vi "test_full_flow.vi"() -> ()   [LabVIEW 2020, in "reqwest_tests.lvlib"]
uses:
  reqwest_tests.lvlib
  <vilib>/addons/_JKI Toolkits/Caraya/classes/Assert/Assert.lvclass
  <vilib>/addons/_JKI Toolkits/Caraya/classes/Test/Test.lvclass
  ClientBuilder/ClientBuilder.lvclass
  Client/Client.lvclass
  Headers/Headers.lvclass
  Request/Request.lvclass
panel:
  out "is_complete":bool
  out "string_value":string
  in  "error in (no error)":errorcluster
  out "error out":errorcluster
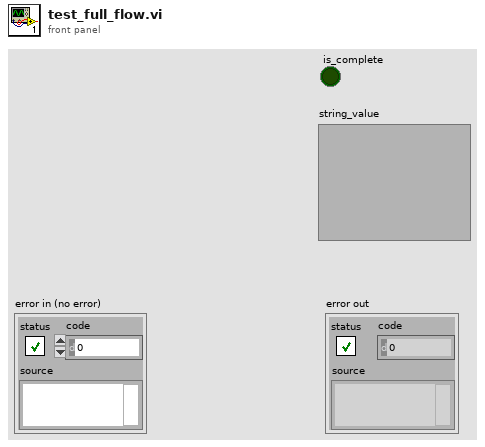
[diagram p1: front panel]
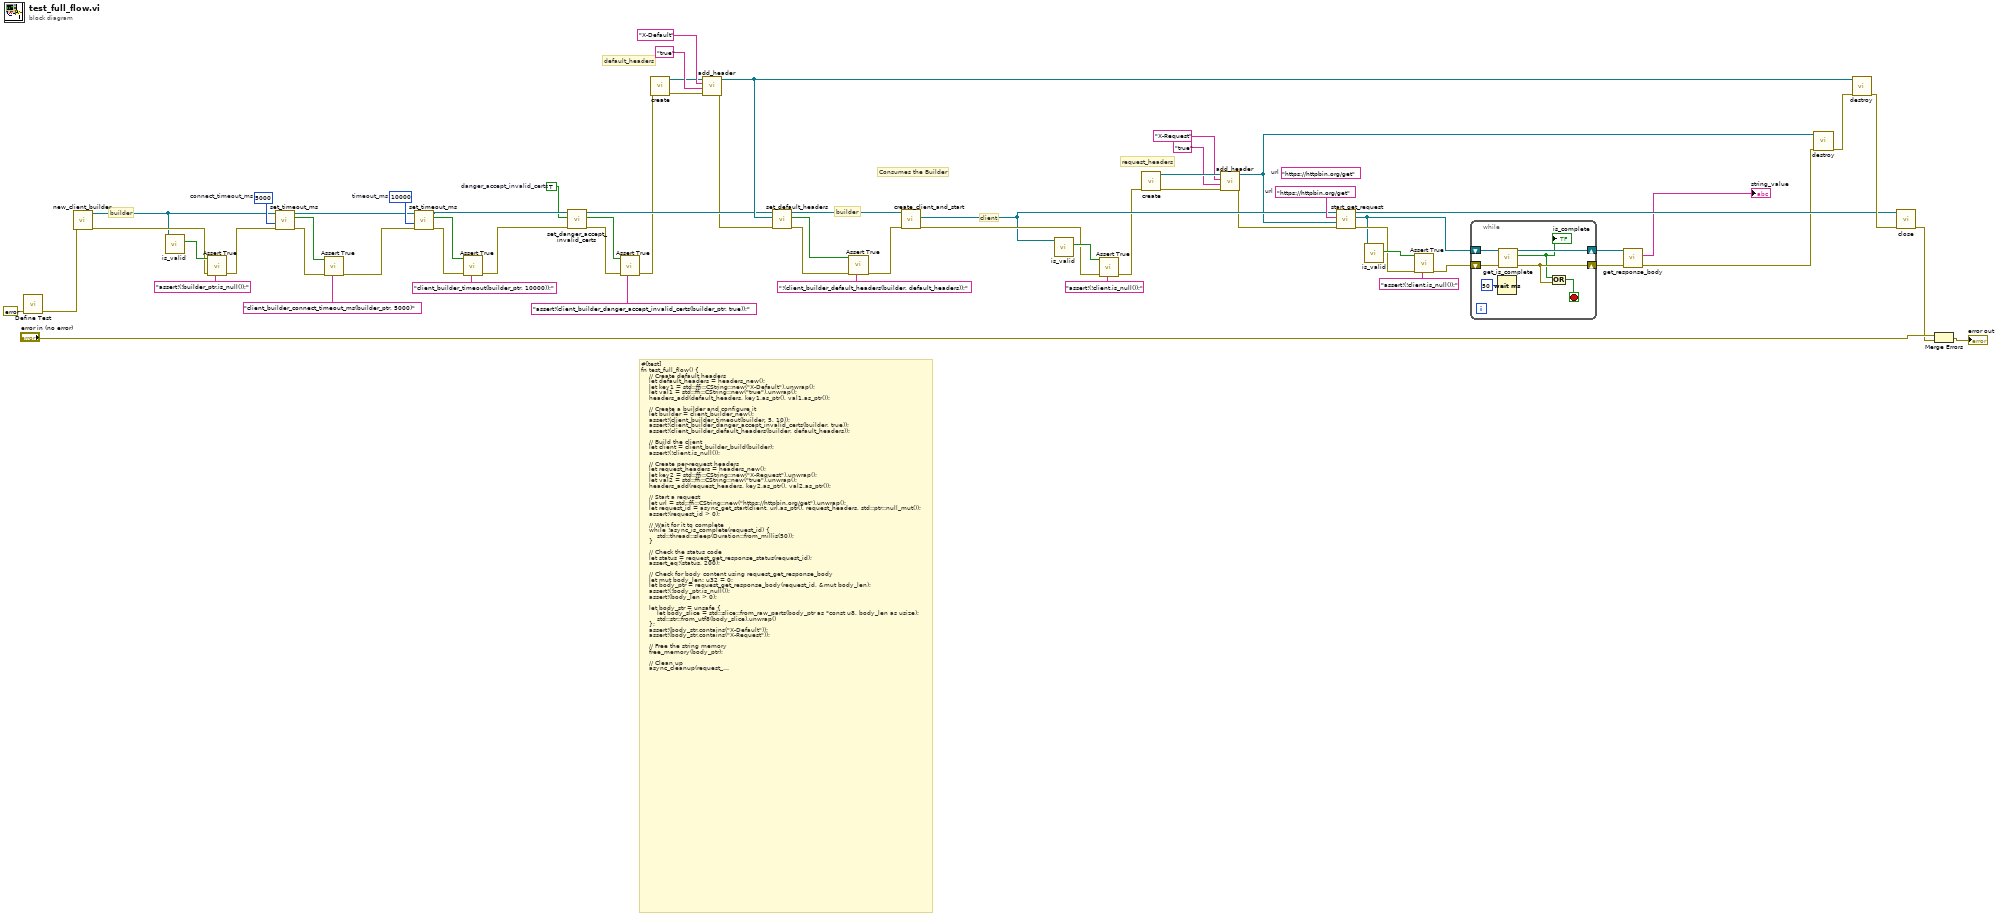
[diagram p0: block diagram]
diagram:
  w5 = u64 5000  # connect_timeout_ms
  (unwired) "https://httpbin.org/get"  # url
  w27 = "https://httpbin.org/get"  # url
  w54 = TRUE  # danger_accept_invalid_certs
  w58 = u64 10000  # timeout_ms
  # "builder"
  # "request_headers"
  # "client"
  # "default_headers"
  # "builder"
  # "Consumes the Builder"
  # "#[test]\nfn test_full_flow() {\n    // Create default headers\n    let default_headers = headers_new();\n    let key1 = std::ffi::CString::new(\"X-Default\").unwrap();\n    let val1 = std::ffi::CString::new(\"true\").unwrap();\n    headers_add(default_headers, key1.as_ptr(), val1.as_ptr());\n\n    // Create a builder and configure it\n    let builder = client_builder_new();\n    assert!(client_builder_timeout(builder, 5, 10));\n    assert!(client_builder_danger_accept_invalid_certs(builder, true));\n    assert!(client_builder_default_headers(builder, default_headers));\n\n    // Build the client\n    let client = client_builder_build(builder);\n    assert!(!client.is_null());\n\n    // Create per-request headers\n    let request_headers = headers_new();\n    let key2 = std::ffi::CString::new(\"X-Request\").unwrap();\n    let val2 = std::ffi::CString::new(\"true\").unwrap();\n    headers_add(request_headers, key2.as_ptr(), val2.as_ptr());\n\n    // Start a request\n    let url = std::ffi::CString::new(\"https://httpbin.org/get\").unwrap();\n    let request_id = async_get_start(client, url.as_ptr(), request_headers, std::ptr::null_mut());\n    assert!(request_id > 0);\n\n    // Wait for it to complete\n    while !async_is_complete(request_id) {\n        std::thread::sleep(Duration::from_millis(50));\n    }\n\n    // Check the status code\n    let status = request_get_response_status(request_id);\n    assert_eq!(status, 200);\n\n    // Check for body content using request_get_response_body\n    let mut body_len: u32 = 0;\n    let body_ptr = request_get_response_body(request_id, &mut body_len);\n    assert!(!body_ptr.is_null());\n    assert!(body_len > 0);\n\n    let body_str = unsafe {\n        let body_slice = std::slice::from_raw_parts(body_ptr as *const u8, body_len as usize);\n        std::str::from_utf8(body_slice).unwrap()\n    };\n    assert!(body_str.contains(\"X-Default\"));\n    assert!(body_str.contains(\"X-Request\"));\n\n    // Free the string memory\n    free_memory(body_ptr);\n\n    // Clean up\n    async_cleanup(request_id);\n    headers_free(request_headers);\n    headers_free(default_headers);\n    client_close(client);\n}"
  n1 = call <vilib>:"Define Test.vi"("error in (no error)"=errorcluster {"status"=FALSE, "code"=0, "source"=""}) -> ("error out"=w48:errorcluster)  [unwired: 9 in, 1 out]
  n2 = call "new_client_builder.vi"("error in (no error)"=w48) -> ("error out"=w47:errorcluster, "Client out"=w4:refnum<class "ClientBuilder.lvclass">)  [unwired: 9 in]
  n3 = call "is_valid.vi"("Client in"=w4) -> ("valid-ref?"=w60:bool)  [unwired: 10 in]
  n4 = call <vilib>:"Assert True.vi"("Label"="assert!(!builder_ptr.is_null());", "error in (no error)"=w47, "True?"=w60) -> ("error out"=w3:errorcluster)  [unwired: 7 in, 1 out]
  n5 = call "set_timeout_ms.vi"("error in (no error)"=w3, "timeout_secs"=w5, "ClientBuilder in"=w4) -> ("error out"=w8:errorcluster, "success"=w7:bool, "ClientBuilder out"=w2:refnum<class "ClientBuilder.lvclass">)  [unwired: 6 in]
  n6 = call <vilib>:"Assert True.vi"("Label"="client_builder_connect_timeout_ms(builder_ptr, 5000)", "error in (no error)"=w8, "True?"=w7) -> ("error out"=w1:errorcluster)  [unwired: 7 in, 1 out]
  n7 = call "set_timeout_ms.vi"("error in (no error)"=w1, "timeout_secs"=w58, "ClientBuilder in"=w2) -> ("error out"=w46:errorcluster, "success"=w56:bool, "ClientBuilder out"=w55:refnum<class "ClientBuilder.lvclass">)  [unwired: 6 in]
  n8 = call <vilib>:"Assert True.vi"("Label"="client_builder_timeout(builder_ptr, 10000));", "error in (no error)"=w46, "True?"=w56) -> ("error out"=w45:errorcluster)  [unwired: 7 in, 1 out]
  n9 = call "set_danger_accept_invalid_certs.vi"("error in (no error)"=w45, "danger_accept_invalid_certs"=w54, "ClientBuilder in"=w55) -> ("error out"=w44:errorcluster, "success"=w52:bool, "ClientBuilder out"=w37:refnum<class "ClientBuilder.lvclass">)  [unwired: 6 in]
  n10 = call <vilib>:"Assert True.vi"("Label"="assert!(client_builder_danger_accept_invalid_certs(builder_ptr, true));", "error in (no error)"=w44, "True?"=w52) -> ("error out"=w21:errorcluster)  [unwired: 7 in, 1 out]
  n11 = call "create.vi"("error in (no error)"=w21) -> ("error out"=w39:errorcluster, "Headers out"=w40:refnum<class "Headers.lvclass">)  [unwired: 9 in]
  n12 = call "add_header.vi"("error in (no error)"=w39, "value"="true", "key"="X-Default", "Headers in"=w40) -> ("error out"=w20:errorcluster, "Headers out"=w38:refnum<class "Headers.lvclass">)  [unwired: 5 in, 1 out]
  n13 = call "set_default_headers.vi"("error in (no error)"=w20, "Headers"=w38, "ClientBuilder in"=w37) -> ("error out"=w34:errorcluster, "success"=w35:bool, "ClientBuilder out"=w36:refnum<class "ClientBuilder.lvclass">)  [unwired: 6 in]
  n14 = call <vilib>:"Assert True.vi"("Label"="!(client_builder_default_headers(builder, default_headers));", "error in (no error)"=w34, "True?"=w35) -> ("error out"=w33:errorcluster)  [unwired: 7 in, 1 out]
  n15 = call "create_client_and_start.vi"("error in"=w33, "ClientBuilder in"=w36) -> ("error out"=w43:errorcluster, "Client out"=w26:refnum<class "Client.lvclass">)  [unwired: 7 in, 1 out]
  n16 = call "is_valid.vi"("Client in"=w26) -> ("valid-ref?"=w51:bool)  [unwired: 10 in]
  n17 = call <vilib>:"Assert True.vi"("Label"="assert!(!client.is_null());", "error in (no error)"=w43, "True?"=w51) -> ("error out"=w17:errorcluster)  [unwired: 7 in, 1 out]
  n18 = call "create.vi"("error in (no error)"=w17) -> ("error out"=w31:errorcluster, "Headers out"=w30:refnum<class "Headers.lvclass">)  [unwired: 9 in]
  n19 = call "add_header.vi"("error in (no error)"=w31, "value"="true", "key"="X-Request", "Headers in"=w30) -> ("error out"=w16:errorcluster, "Headers out"=w22:refnum<class "Headers.lvclass">)  [unwired: 5 in, 1 out]
  n20 = call "start_get_request.vi"("error in (no error)"=w16, "Headers in"=w22, "url"=w27, "Client in"=w26) -> ("error out"=w23:errorcluster, "Request"=w14:refnum<class "Request.lvclass">, "Client out"=w15:refnum<class "Client.lvclass">)  [unwired: 5 in]
  n21 = call "is_valid.vi"("Request in"=w14) -> ("valid-ref?"=w24:bool)  [unwired: 10 in]
  n22 = call <vilib>:"Assert True.vi"("Label"="assert!(!client.is_null());", "error in (no error)"=w23, "True?"=w24) -> ("error out"=w13:errorcluster)  [unwired: 7 in, 1 out]
  n23 = while {
    shift-right: [w70] -> w9
    shift-left: w14 -> [w69]
    shift-right: [w66] -> w12
    shift-left: w13 -> [w67]
    stop <- w64 stop-if-true
    n24 = Wait (ms)(milliseconds to wait=u32 50) -> ()  [unwired: 1 out]
    n25 = call "get_is_complete.vi"("error in (no error)"=w67, "Request in"=w69) -> ("error out"=w66:errorcluster, "is_complete"=w65:bool, "Request out"=w70:refnum<class "Request.lvclass">)  [unwired: 7 in]
    "is_complete" <- w65
    n26 = Or(x=w65, y=w66) -> (x .or. y?=w64:bool)
  }
  n27 = call "get_response_body.vi"("error in (no error)"=w12, "Request in"=w9) -> ("error out"=w11:errorcluster, "string_value"=→"string_value":string)  [unwired: 7 in, 1 out]
  n28 = call "destroy.vi"("error in (no error)"=w11, "Headers in"=w22) -> ("error out"=w19:errorcluster)  [unwired: 9 in]
  n29 = call "destroy.vi"("error in (no error)"=w19, "Headers in"=w38) -> ("error out"=w18:errorcluster)  [unwired: 9 in]
  n30 = call "close.vi"("error in (no error)"=w18, "Client in"=w15) -> ("error out"=w49:errorcluster)  [unwired: 9 in]
  n31 = Merge Errors("error in (no error)", w49) -> (→"error out":errorcluster)
